vi "Subset (multiple).vi"(8 "error in (no error)":errorcluster, 9 "Subset Method":enum16{"Slider (%)", "X[] min and max"}(ring)=enum."X[] min and max", 10 "Subset Slider":cluster{dbl, dbl}(slide)={75.0, 25.0} scale=0.0..100.0 scale format="%#_6f", 11 "XY-data":cluster{"X-array":dbl[], "Y-array":dbl[]}[](array[cluster]) {"Y-array" format="%.2p"; "X-array" format="%.2p"}) -> (0 "error out":errorcluster, 3 "Subset XY-data out":cluster{"X-array":dbl[], "Y-array":dbl[]}[](array[cluster]) {"Y-array" format="%.2p"; "X-array" format="%.2p"})   [LabVIEW 2019, in "xy_utilities.lvlib"]
doc: "Returns a subset of <b>XY-data</b>\n\n<b>Subset Method</b>: choose how to define the subset.\n- <b>X[] min and max</b>: returns subset of data between found maximum and minimum values of <b>x-array</b>. Returns data in ascending x order.\n- <b>Slider (%)</b>: chooses data subset based on percentages (%) defined by <b>Subset Slider</b> \n\nWire data to the data input to determine the polymorphic instance to use or manually select the instance."
uses:
  xy_utilities.lvlib
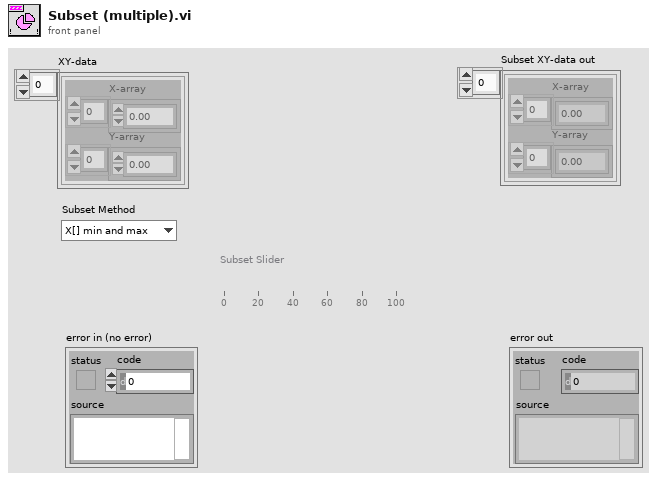
[diagram p1: front panel]
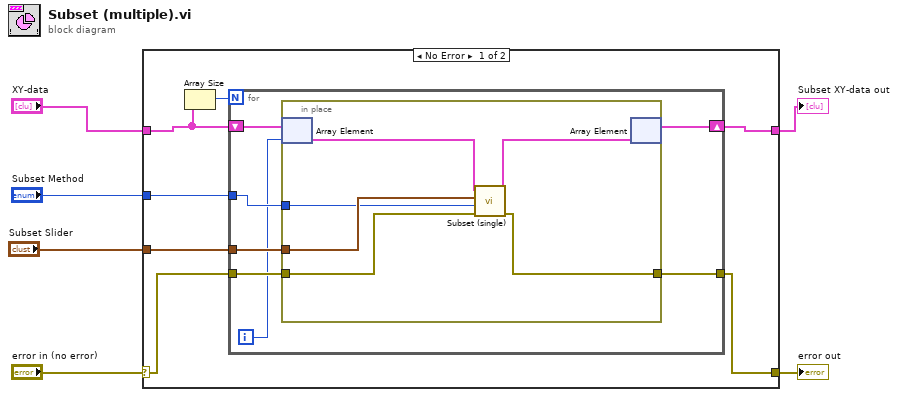
[diagram p0: block diagram]
diagram:
  n1 = case shown="No Error" "error in (no error)" {
    selector: "error in (no error)" -> [w10 w28]
    tunnel: [w9 w28] -> w5
    tunnel: "XY-data" -> [w7 w27]
    tunnel: [w11 w27] -> w3
    tunnel: "Subset Method" -> [w12 _]
    tunnel: "Subset Slider" -> [w13 _]
    frame No Error {
      n2 = Array Size(array=w7) -> (size(s)=w8:i32)
      n3 = for {
        N: w8 -> [_]
        tunnel: w13 -> [w20]
        tunnel: w12 -> [w19]
        tunnel: w10 -> [w18]
        tunnel: [w17] -> w9
        shift-right: [w14] -> w11
        shift-left: w7 -> [w16]
        i -> [w15]
        n4 = in-place {
          in-place-border: w20 -> [w26]
          in-place-border: w19 -> [w25]
          in-place-border: w18 -> [w24]
          in-place-border: [w23] -> w17
          n5 = in-place-array #1(w16, w15) -> (w22:cluster{"X-array":dbl[], "Y-array":dbl[]})
          n6 = call "Subset (single).vi"("error in (no error)"=w24, "Subset Method"=w25, "Subset Slider (%)"=w26, "XY-data"=w22) -> ("error out"=w23:errorcluster, "XY-data out"=w21:cluster{"X-array":dbl[], "Y-array":dbl[]})  [unwired: 6 in]
          n7 = in-place-array #1(w21) -> (w14:cluster{"X-array":dbl[], "Y-array":dbl[]}[])  [unwired: 1 out]
        }
      }
    }
    frame Error {
    }
  }
  "error out" <- w5
  "Subset XY-data out" <- w3
